vi "Acq_Read.vi"(8 "error in (no error)":errorcluster, 10 "rt fifo ref in":refnum<k33>, 11 "Refnum in":refnum<k20>) -> (0 "error out":errorcluster, 1 "Array":i16[][](array[numeric]), 2 "rt fifo ref out":refnum<k33>, 3 "Refnum out":refnum<k20>, 5 "Elements Remaining":u32)   [LabVIEW 2025]
uses:
  <vilib>/rvi/interface/nirviMethod/nirviMethod.xnode
  <vilib>/FPGAPlugInAG/Dynamic/niLvFpga_ReadFifo_Dynamic.vi
  <vilib>/rvi/errors/niLvFpgaMergeErrorWithErrorCode.vi
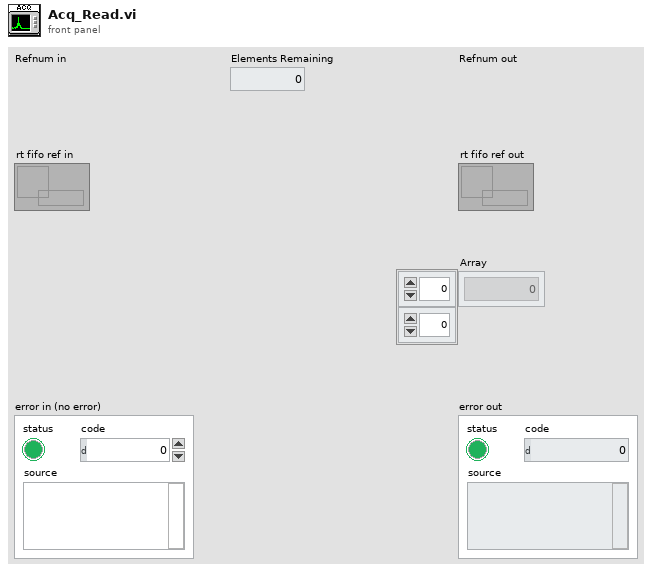
[diagram p1: front panel]
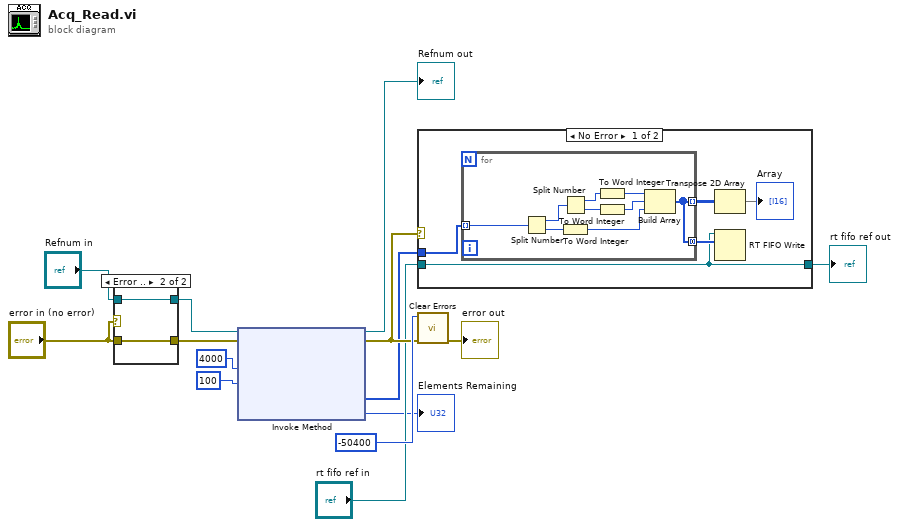
[diagram p0: block diagram]
diagram:
  n1 = case shown="Error .." "error in (no error)" {
    tunnel: "Refnum in" -> [w16 w18]
    tunnel: [w16 w18] -> w1
    tunnel: "error in (no error)" -> [w15 w17]
    tunnel: [w15 w17] -> w2
    frame No Error {
    }
    frame Error {
    }
  }
  n2 = xnode "Invoke Method"("FPGA VI Reference In"=w1, "error in"=w2, "Number of Elements"=u32 4000, "Timeout (ms)"=100) -> ("FPGA VI Reference Out"=→"Refnum out":refnum<k20>, "error out"=w11:errorcluster, "Data"=w8:u64[], "Elements Remaining"=→"Elements Remaining":u32)
  n3 = case shown="No Error" w11 {
    tunnel: w8 -> [w23 _]
    tunnel: "rt fifo ref in" -> [w20 w33]
    tunnel: [w20 w33] -> w14
    frame No Error {
      n4 = for {
        tunnel: w23 -> [w32] mode=indexing
        tunnel: [w24] -> w22 mode=concatenating
        tunnel: [w24] -> w21 mode=indexing
        n5 = Split Number(x=w32) -> (hi(x)=w31:u32, lo(x)=w28:u32)
        n6 = To Word Integer(number=w28) -> (16bit integer=w25:i16)
        n7 = Split Number(x=w31) -> (hi(x)=w30:u16, lo(x)=w29:u16)
        n8 = To Word Integer(number=w30) -> (16bit integer=w27:i16)
        n9 = To Word Integer(number=w29) -> (16bit integer=w26:i16)
        n10 = Build Array(w27, w26, w25) -> (w24:i16[])
      }
      n11 = Transpose 2D Array(2D array=w21) -> (transposed array=→"Array":i16[][])
      n12 = RT FIFO Write(0:w20, 1:w22) -> ()  [unwired: 3 in, 4 out]
    }
    frame Error {
    }
  }
  "rt fifo ref out" <- w14
  n13 = call <vilib>:"Clear Errors.vi"("error in (no error)"=w11, "specific error code to clear (0: all)"=-50400) -> ("error out"=→"error out":errorcluster)  [unwired: 4 in, 1 out]
